vi "Overlay_Blit.vi"(0 "Picture":u8[][](array[numeric]), 5 "Sprites":cluster{"Pix":u8[][], "Mask":u8[][]}[](array[cluster]), 7 "State":T2={"Tick"=0, "Phase"=0, "PhaseTicks"=0, "Level"=1, "Room"=0, "X10"=0, "Y10"=0, "VY10"=0, "Mode"=0, "Facing"=0, "Run"=0, "Vert"=0, "StandY"=0, "EntryX10"=0, "EntryY10"=0, "EntryMode"=0, "Lives"=4, "Score"=0, "NextLife"=10000, "KeyR"=0, "KeyB"=0, "KeyY"=0, "Torch"=FALSE, "FloorPhase"=0, "Dead"=FALSE, "LevelStart"=FALSE, "Quit"=FALSE, "Sound"=0, "Seed"=12345, "DemoStep"=0, "Tiles"=[], "World"=[], "Enemies"=[], "Highscores"=[], "Name"=[0, 0, 0], "Cursor"=0}, 9 "Clip":T1={"left"=0, "top"=0, "right"=1280, "bottom"=720}, 11 "error in":errorcluster) -> (4 "Picture out":u8[][](array[numeric]), 15 "error out":errorcluster)   [LabVIEW 2020, in "GH_Render.lvlib"]
doc: "Draws the message of the phase on top: highscore table (title), DEMO - PRESS ENTER, LEVEL n / READY, PAUSE, TREASURE!, LEVEL CLEAR, GAME OVER and the name entry. Only when its box meets Clip (screen pixels)."
uses:
  GH_Render.lvlib
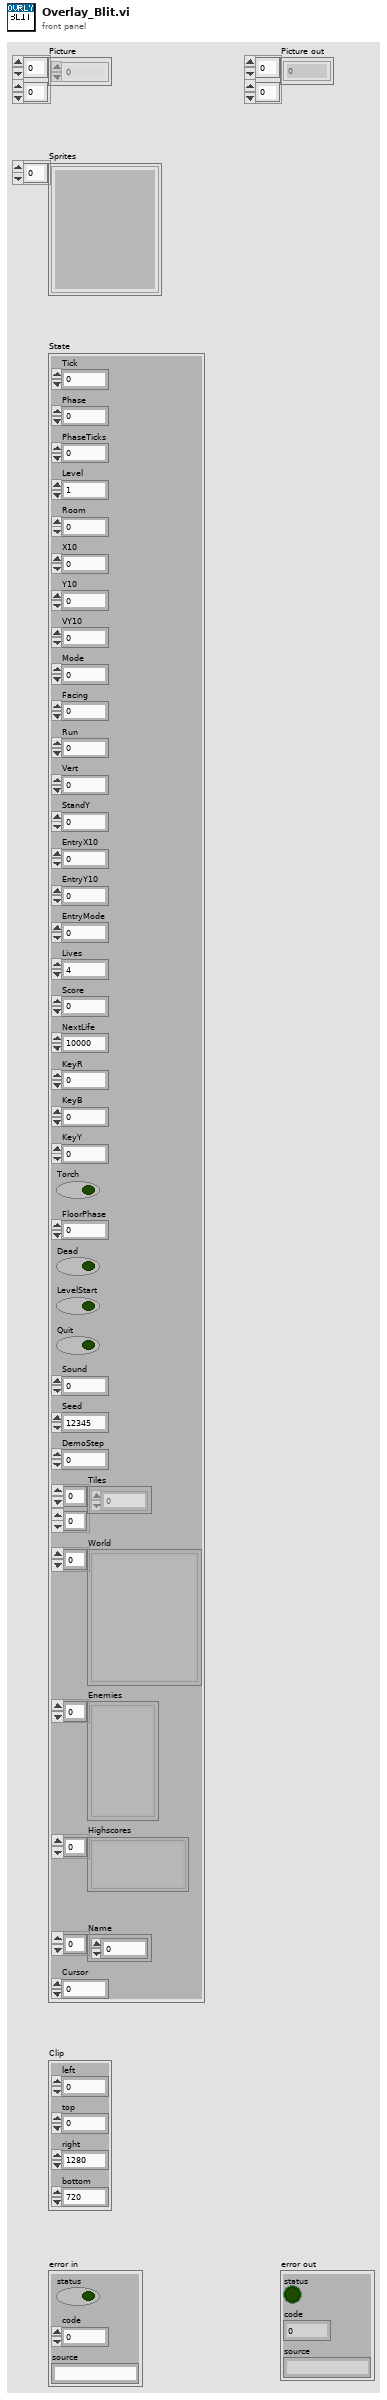
[diagram p1: front panel]
types:
  T1 = cluster{"left":i16, "top":i16, "right":i16, "bottom":i16}
  T2 = cluster{"Tick":u32, "Phase":i32, "PhaseTicks":i32, "Level":i32, "Room":i32, "X10":i32, "Y10":i32, "VY10":i32, "Mode":i32, "Facing":i32, "Run":i32, "Vert":i32, "StandY":i32, "EntryX10":i32, "EntryY10":i32, "EntryMode":i32, "Lives":i32, "Score":i32, "NextLife":i32, "KeyR":i32, "KeyB":i32, "KeyY":i32, "Torch":bool, "FloorPhase":i32, "Dead":bool, "LevelStart":bool, "Quit":bool, "Sound":i32, "Seed":u32, "DemoStep":i32, "Tiles":u8[][], "World":cluster{"ID":string, "Depth":i32, "Column":i32, "Tiles":u8[][]}[], "Enemies":cluster{"Kind":i32, "X10":i32, "Y10":i32, "Dir":i32, "Mode":i32}[], "Highscores":cluster{"Score":i32, "Name":string}[], "Name":i32[], "Cursor":i32}
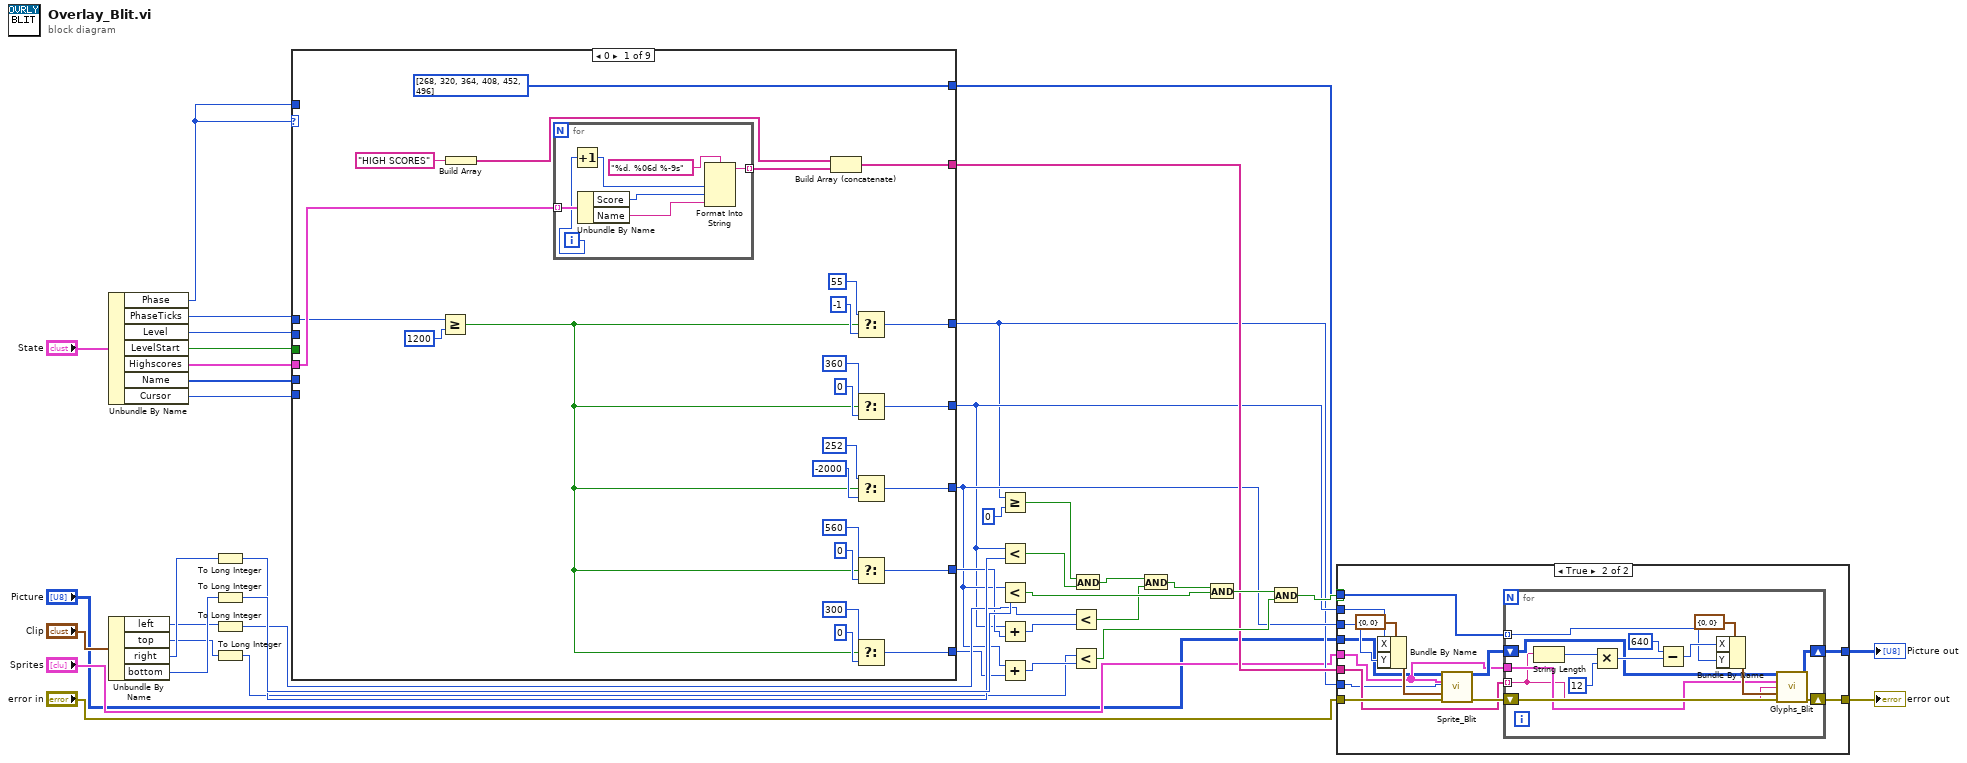
[diagram p0: block diagram]
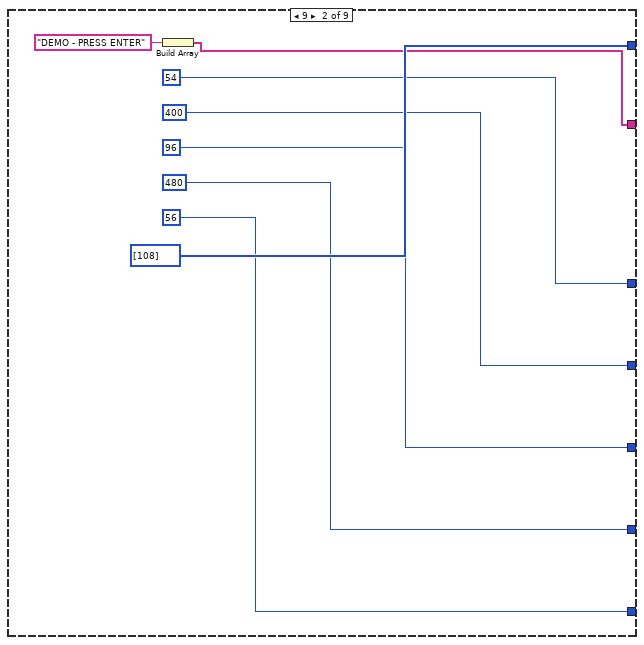
[diagram p3: hidden frame]
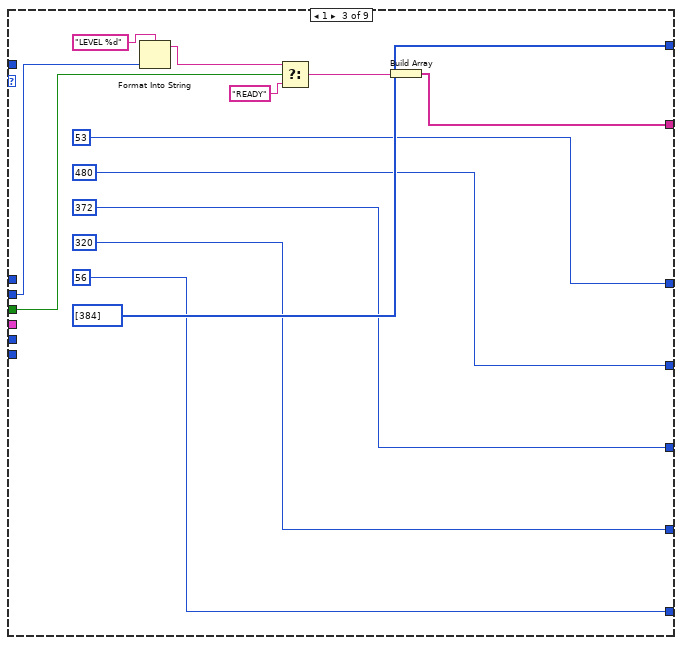
[diagram p4: hidden frame]
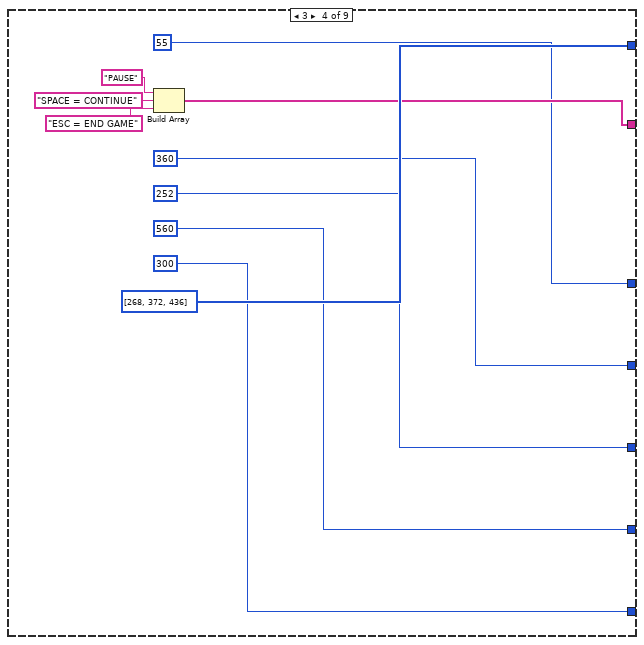
[diagram p5: hidden frame]
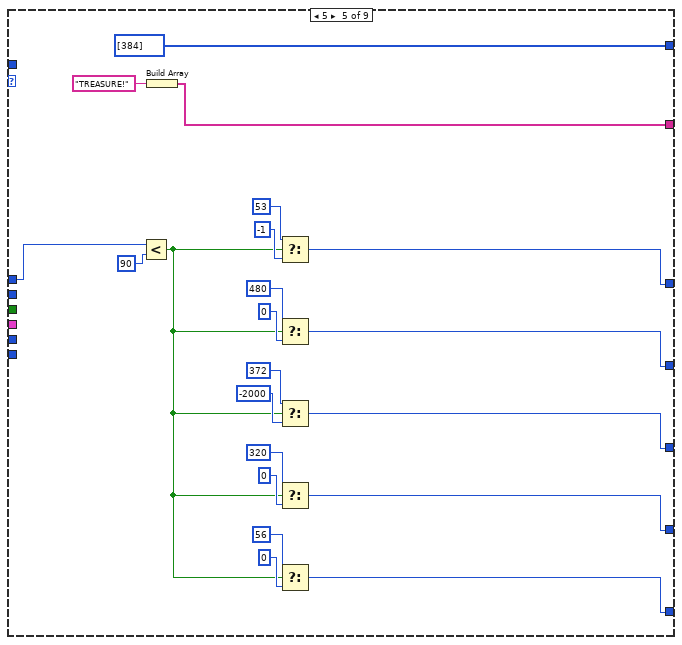
[diagram p6: hidden frame]
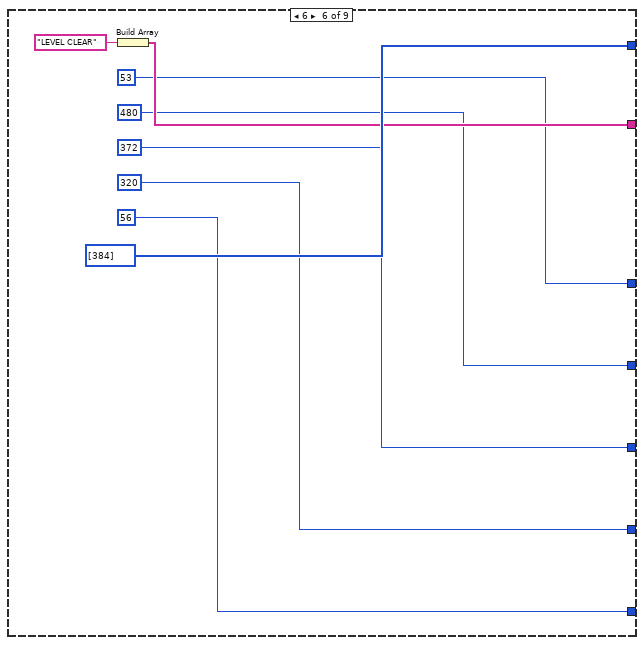
[diagram p7: hidden frame]
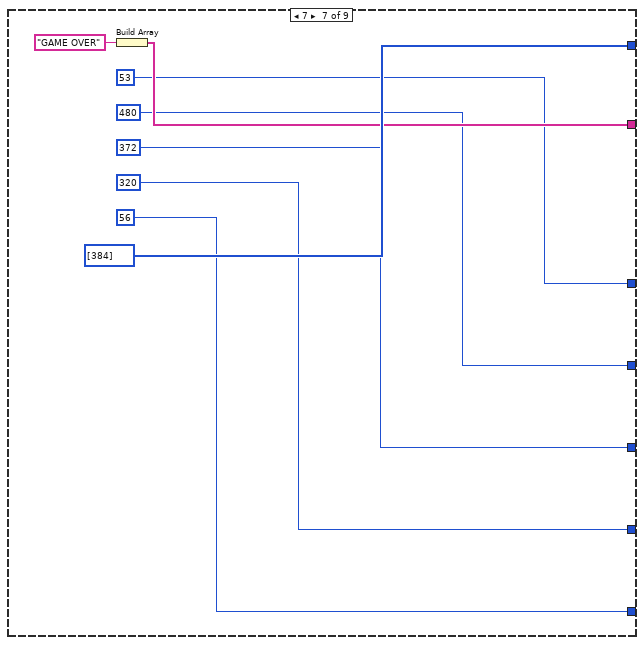
[diagram p8: hidden frame]
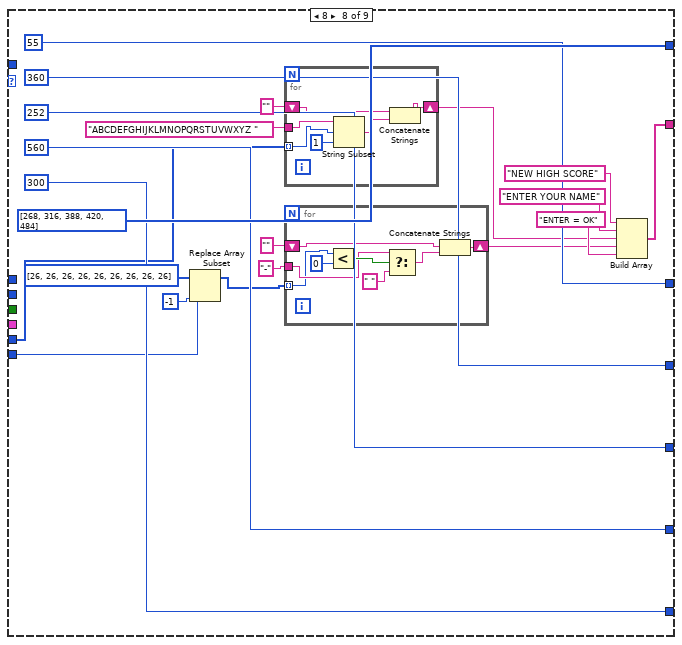
[diagram p9: hidden frame]
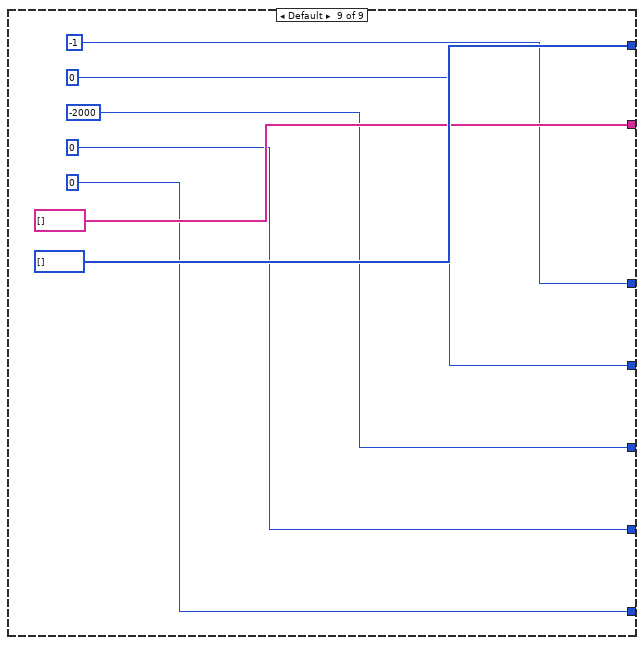
[diagram p10: hidden frame]
diagram:
  n1 = Unbundle By Name("State") -> ("Phase"=w6:i32, "PhaseTicks"=w7:i32, "Level"=w8:i32, "LevelStart"=w9:bool, "Highscores"=w10:cluster{"Score":i32, "Name":string}[], "Name"=w11:i32[], "Cursor"=w12:i32)
  n2 = Unbundle By Name("Clip") -> ("left"=w20:i16, "top"=w21:i16, "right"=w22:i16, "bottom"=w23:i16)
  n3 = To Long Integer(number=w22) -> (32bit integer=w26:i32)
  n4 = To Long Integer(number=w23) -> (32bit integer=w27:i32)
  n5 = To Long Integer(number=w20) -> (32bit integer=w24:i32)
  n6 = To Long Integer(number=w21) -> (32bit integer=w25:i32)
  n7 = case shown="0" w6 {
    tunnel: [i32[] [268, 320, 364, 408, 452, 496] ("Line y") i32[] [108] ("Line y") i32[] [384] ("Line y") i32[] [268, 372, 436] ("Line y") i32[] [384] ("Line y") i32[] [384] ("Line y") i32[] [384] ("Line y") i32[] [268, 316, 388, 420, 484] ("Line y") i32[] []] -> w19
    tunnel: w6 -> [_ _ _ _ _ _ _ _ _]
    tunnel: w7 -> [w42 _ _ _ w104 _ _ _ _]
    tunnel: w10 -> [w43 _ _ _ _ _ _ _ _]
    tunnel: w9 -> [_ _ w81 _ _ _ _ _ _]
    tunnel: w8 -> [_ _ w82 _ _ _ _ _ _]
    tunnel: w11 -> [_ _ _ _ _ _ _ w141 _]
    tunnel: w12 -> [_ _ _ _ _ _ _ w142 _]
    tunnel: [w53 54 53 55 w109 53 53 55 -1] -> w13
    tunnel: [w56 400 480 360 w112 480 480 360 0] -> w14
    tunnel: [w59 96 372 252 w115 372 372 252 -2000] -> w15
    tunnel: [w62 480 320 560 w118 320 320 560 0] -> w16
    tunnel: [w65 56 56 300 w121 56 56 300 0] -> w17
    tunnel: [w49 w79 w92 w102 w123 w131 w139 w160 string[] []] -> w18
    frame 0 {
      n8 = Greater Or Equal?(x=w42, y=1200) -> (x >= y?=w45:bool)
      n9 = Build Array("HIGH SCORES") -> (w48:string[])
      n10 = for {
        tunnel: w43 -> [w67] mode=indexing
        tunnel: [w72] -> w46 mode=indexing
        i -> [w66]
        n11 = Increment(x=w66) -> (x+1=w70:i32)
        n12 = Unbundle By Name(w67) -> ("Score"=w68:i32, "Name"=w69:string)
        n13 = Format Into String(format string="%d. %06d %-9s", w70, w68, w69) -> (resulting string=w72:string)  [unwired: 2 in, 1 out]
      }
      n14 = Build Array (concatenate)(w48, w46) -> (w49:string[])
      n15 = Select(t=55, s=w45, f=-1) -> (s? t:f=w53:i32)
      n16 = Select(t=360, s=w45, f=0) -> (s? t:f=w56:i32)
      n17 = Select(t=252, s=w45, f=-2000) -> (s? t:f=w59:i32)
      n18 = Select(t=560, s=w45, f=0) -> (s? t:f=w62:i32)
      n19 = Select(t=300, s=w45, f=0) -> (s? t:f=w65:i32)
    }
    frame 9 {
      n20 = Build Array("DEMO - PRESS ENTER") -> (w79:string[])
    }
    frame 1 {
      n21 = Format Into String(format string="LEVEL %d", w82) -> (resulting string=w84:string)  [unwired: 2 in, 1 out]
      n22 = Select(t=w84, s=w81, f="READY") -> (s? t:f=w86:string)
      n23 = Build Array(w86) -> (w92:string[])
    }
    frame 3 {
      n24 = Build Array("PAUSE", "SPACE = CONTINUE", "ESC = END GAME") -> (w102:string[])
    }
    frame 5 {
      n25 = Less?(x=w104, y=90) -> (x < y?=w106:bool)
      n26 = Build Array("TREASURE!") -> (w123:string[])
      n27 = Select(t=53, s=w106, f=-1) -> (s? t:f=w109:i32)
      n28 = Select(t=480, s=w106, f=0) -> (s? t:f=w112:i32)
      n29 = Select(t=372, s=w106, f=-2000) -> (s? t:f=w115:i32)
      n30 = Select(t=320, s=w106, f=0) -> (s? t:f=w118:i32)
      n31 = Select(t=56, s=w106, f=0) -> (s? t:f=w121:i32)
    }
    frame 6 {
      n32 = Build Array("LEVEL CLEAR") -> (w131:string[])
    }
    frame 7 {
      n33 = Build Array("GAME OVER") -> (w139:string[])
    }
    frame 8 {
      n34 = Replace Array Subset(array=i32[] [26, 26, 26, 26, 26, 26, 26, 26, 26], new element=-1, index=w142) -> (w148:i32[])
      n35 = for {
        tunnel: "ABCDEFGHIJKLMNOPQRSTUVWXYZ " -> [w171]
        shift-right: [w173] -> w145
        shift-left: "" -> [w172]
        tunnel: w141 -> [w170] mode=indexing
        n36 = String Subset(string=w171, offset (0)=w170, length (rest)=1) -> (substring=w175:string)
        n37 = Concatenate Strings(w172, w175) -> (w173:string)
      }
      n38 = for {
        tunnel: "-" -> [w163]
        shift-right: [w165] -> w151
        shift-left: "" -> [w164]
        tunnel: w148 -> [w162] mode=indexing
        n39 = Less?(x=w162, y=0) -> (x < y?=w167:bool)
        n40 = Select(t=w163, s=w167, f=" ") -> (s? t:f=w169:string)
        n41 = Concatenate Strings(w164, w169) -> (w165:string)
      }
      n42 = Build Array("NEW HIGH SCORE", "ENTER YOUR NAME", w145, w151, "ENTER = OK") -> (w160:string[])
    }
    frame Default {
    }
  }
  n43 = Greater Or Equal?(x=w13, y=0) -> (x >= y?=w29:bool)
  n44 = Less?(x=w14, y=w26) -> (x < y?=w30:bool)
  n45 = Less?(x=w15, y=w27) -> (x < y?=w33:bool)
  n46 = Add(x=w14, y=w16) -> (x+y=w31:i32)
  n47 = Add(x=w15, y=w17) -> (x+y=w34:i32)
  n48 = Less?(x=w24, y=w31) -> (x < y?=w32:bool)
  n49 = Less?(x=w25, y=w34) -> (x < y?=w35:bool)
  n50 = And(x=w29, y=w30) -> (x .and. y?=w36:bool)
  n51 = And(x=w36, y=w32) -> (x .and. y?=w37:bool)
  n52 = And(x=w37, y=w33) -> (x .and. y?=w38:bool)
  n53 = And(x=w38, y=w35) -> (x .and. y?=w39:bool)
  n54 = case shown="True" w39 {
    tunnel: "Picture" -> [w183 w185]
    tunnel: "Sprites" -> [_ w186]
    tunnel: "error in" -> [w184 w192]
    tunnel: w19 -> [_ w191]
    tunnel: w13 -> [_ w187]
    tunnel: w14 -> [_ w188]
    tunnel: w15 -> [_ w189]
    tunnel: w18 -> [_ w190]
    tunnel: [w183 w197] -> w40
    tunnel: [w184 w198] -> w41
    frame False {
    }
    frame True {
      n55 = Bundle By Name(cluster=cluster{"X":i32, "Y":i32} {"X"=0, "Y"=0}, "X"=w188, "Y"=w189) -> (w194:cluster{"X":i32, "Y":i32})
      n56 = call "Sprite_Blit.vi"("Picture"=w185, "Sprites"=w186, "Index"=w187, "Position"=w194, "error in"=w192) -> ("Picture out"=w195:u8[][], "error out"=w196:errorcluster)  [unwired: 9 in]
      n57 = for {
        tunnel: w186 -> [w201]
        tunnel: w191 -> [w200] mode=indexing
        shift-right: [w203] -> w197
        shift-left: w195 -> [w202]
        shift-right: [w205] -> w198
        shift-left: w196 -> [w204]
        tunnel: w190 -> [w199] mode=indexing
        n58 = String Length(string=w199) -> (length=w206:i32)
        n59 = Multiply(x=w206, y=12) -> (x*y=w209:i32)
        n60 = Subtract(x=640, y=w209) -> (x-y=w210:i32)
        n61 = Bundle By Name(cluster=cluster{"X":i32, "Y":i32} {"X"=0, "Y"=0}, "X"=w210, "Y"=w200) -> (w212:cluster{"X":i32, "Y":i32})
        n62 = call "Glyphs_Blit.vi"("Picture"=w202, "Sprites"=w201, "Text"=w199, "Position"=w212, "error in"=w204) -> ("Picture out"=w203:u8[][], "error out"=w205:errorcluster)  [unwired: 9 in]
      }
    }
  }
  "Picture out" <- w40
  "error out" <- w41
